vi "Measurement UI.vi"() -> ()   [LabVIEW 2021, in "Load Transient Response_PMIC.lvlib"]
uses:
  Load Transient Response_PMIC.lvlib
panel:
  in  "MeasGraphs":enum32{"LOAD TRANSIENT", "Hidden Controls"}(tab)
  out "MeasTable":string[][](table)
  out "LoadCurrentV/STimeGraph":waveform(dbl)(graph) caption="Load Transient"
  out "OutputVoltageV/STimeGraph":waveform(dbl)(graph) caption="Load Transient"
  in  "Load Current v/s Time":string="LOAD CURRENT vs TIME"
  in  "Output Voltage v/s Time":string="LOAD VOLTAGE vs TIME"
  out "Overshoot load voltage":dbl
  out "Undershoot load voltage":dbl
  in  "Source resource name":string
  in  "Load resource name":string
  out "dt":dbl
  out "Load voltages":dbl[](array[numeric])
  out "Load currents":dbl[](array[numeric])
  in  "Source transient response":i32(ring)=1042 items=["Slow"=1041, "Normal"=1038, "Fast"=1039, "Custom"=1042]
  in  "Load transient response":i32(ring)=3 items=["Slow"=1041, "Normal"=1038, "Fast"=1039, "Custom"=1042]
  in  "Load sense":i32(ring)=1009 caption="SENSE" items=["Local"=1008, "Remote"=1009]
  in  "Source sense":i32(ring)=1009 caption="SENSE" items=["Local"=1008, "Remote"=1009]
  in  "Load current delay t2":dbl=0.001 caption="DELAY T2" format="%#_6ps"
  in  "Load current delay t1":dbl=0.001 caption="DELAY T1" format="%#_6ps"
  in  "Load current pulse duration":dbl=0.001 caption="PULSE DURATION" format="%#_6ps"
  in  "Load current level range":dbl=40.0 caption="CURRENT LEVEL RANGE" format="%#_6pA"
  in  "Load current rising slew rate":dbl=24.0 caption="CURRENT RISING SLEW RATE" format="%#_6pA/us"
  in  "Load current falling slew rate":dbl=24.0 caption="CURRENT FALLING SLEW RATE" format="%#_6pA/us"
  in  "Load configuration":string="Load configuration"
  in  "Source configuration":string="Source configuration"
  in  "Source voltage level":dbl=12.0 caption="VOLTAGE LEVEL" format="%#_6pV"
  in  "Source current limit":dbl=25.0 caption="CURRENT LIMIT" format="%#_6pA"
  in  "PPSResourceName":refnum<k15> caption="RESOURCE NAME"
  in  "Source voltage pole-zero ratio":dbl=2.0 caption="POLE-ZERO RATIO"
  in  "Source voltage gain bandwidth":dbl=2000.0 caption="GAIN BANDWIDTH" format="%#_6pHz"
  in  "Source voltage compensation frequency":dbl=3530.0 caption="COMP. FREQUENCY" format="%#_6pHz"
  in  "Source fast":bool
  in  "Source normal":bool
  in  "Source slow":bool
  in  "Source SourceAdapt":string="Voltage SourceAdapt Parameters"
  in  "Load voltage limit range":dbl=6.0 caption="VOLTAGE LIMIT RANGE" format="%#_6pV"
  in  "Load current set point 1":dbl=4.0 caption="CURRENT SET POINT 1" format="%#_6pA"
  in  "Load current pole-zero ratio":dbl=0.3 caption="POLE-ZERO RATIO"
  in  "Load current gain bandwidth":dbl=14000.0 caption="GAIN BANDWIDTH" format="%#_6pHz"
  in  "Load current compensation frequency":dbl=180000.0 caption="COMP. FREQUENCY" format="%#_6pHz"
  in  "Load sample rate":dbl=1800000.0 caption="SAMPLE RATE" format="%#_6pS/s"
  in  "Load current set point 2":dbl=14.0 caption="CURRENT SET POINT 2" format="%#_6pA"
  in  "ELOADResourceName":refnum<k15> caption="RESOURCE NAME"
  in  "Load fast":bool
  in  "Load normal":bool
  in  "Load slow":bool
  in  "Load SourceAdapt":string="Current SourceAdapt Parameters"
  out "Status":string
  in  "DUT setup time":dbl=1.0 caption="DUT SETUP TIME" format="%#_6ps"
  in  "Measurement settings":string="Measurement settings"
  in  "Nominal output voltage":dbl=3.3 caption="NOMINAL OUTPUT VOLTAGE" format="%#_6pV"
  in  "Mode of operation":T1(ring)=enum."Perform measurement" caption="MODE OF OPERATION"
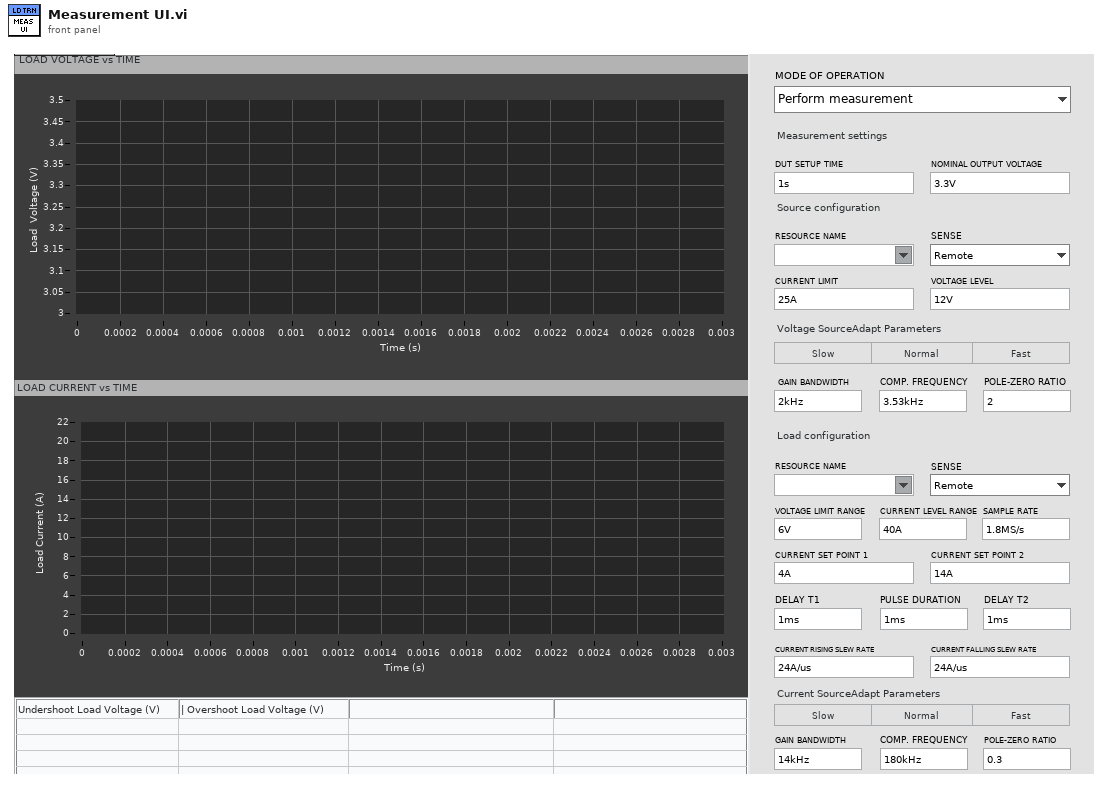
[diagram p1: front panel]
types:
  T1 = enum32{"Power on the DUT", "Perform measurement", "Power off the DUT"}
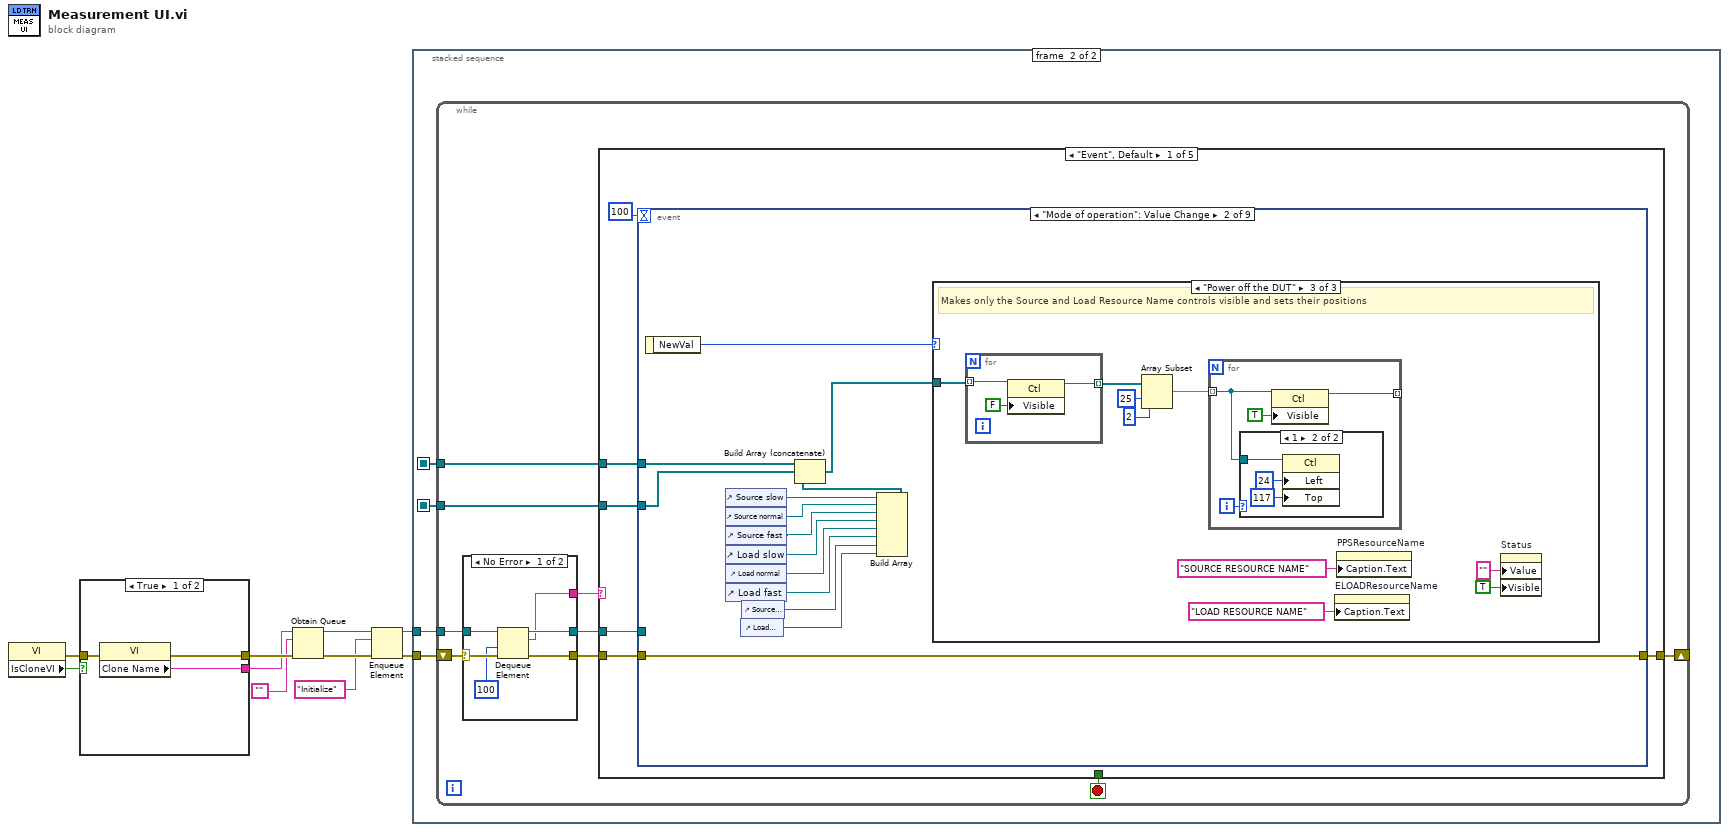
[diagram p0: block diagram]
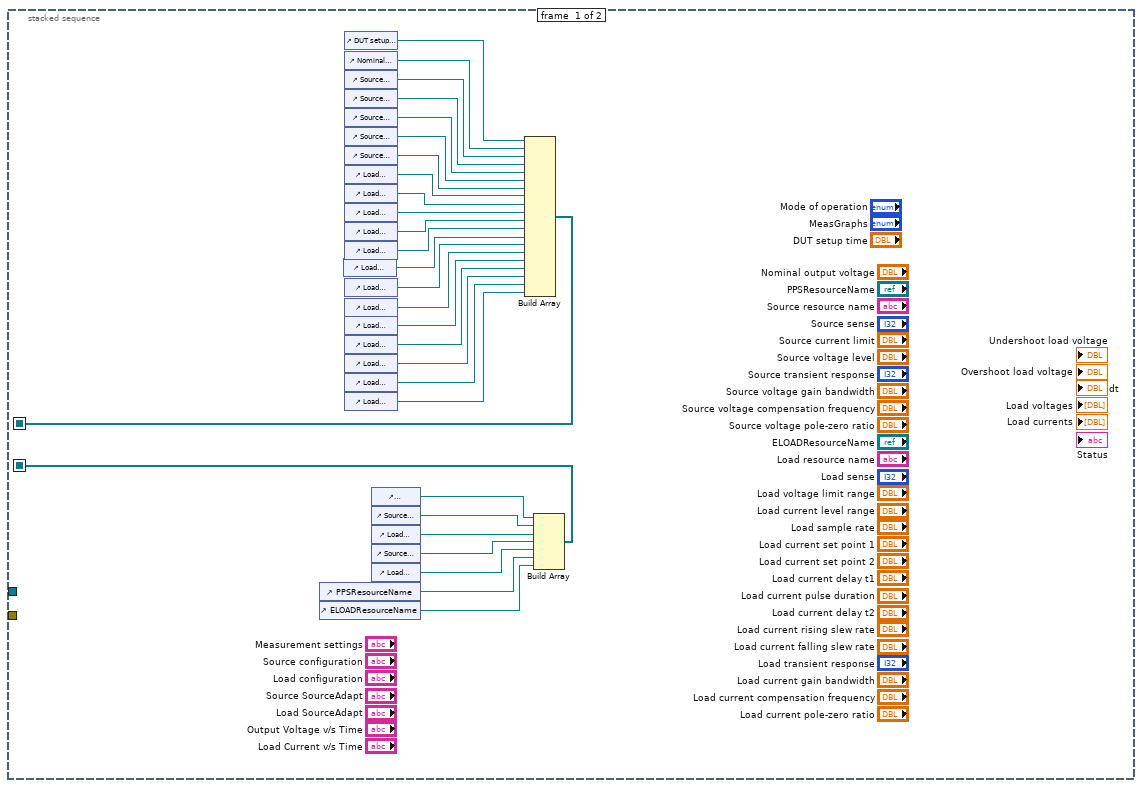
[diagram p2: hidden frame]
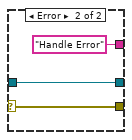
[diagram p3: hidden frame]
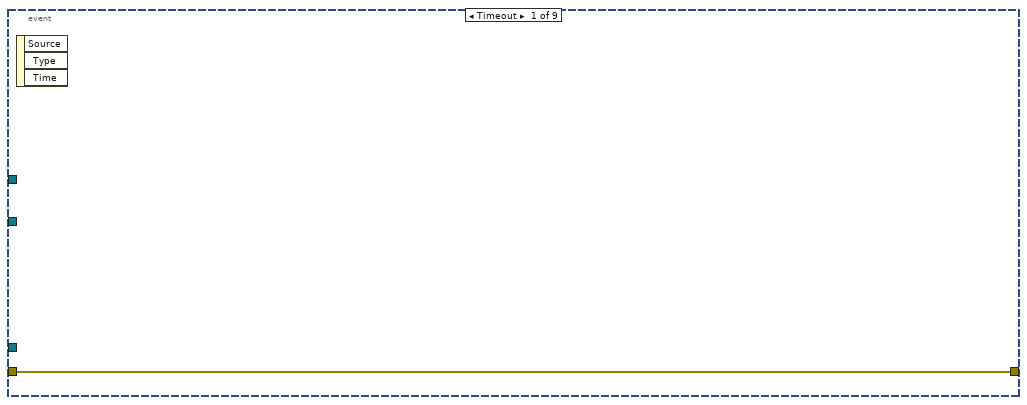
[diagram p4: hidden frame]
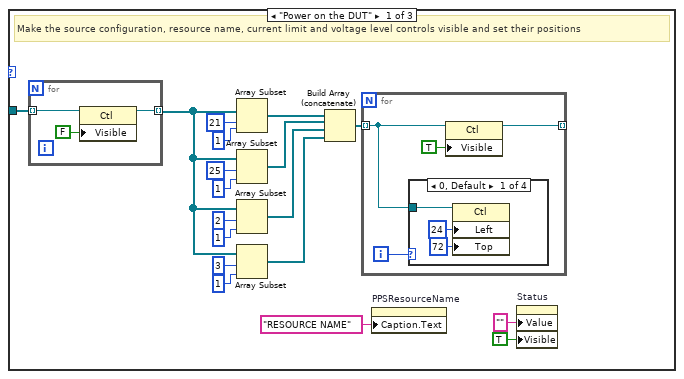
[diagram p5: hidden frame]
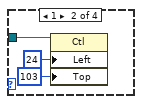
[diagram p6: hidden frame]
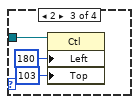
[diagram p7: hidden frame]
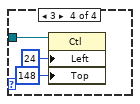
[diagram p8: hidden frame]
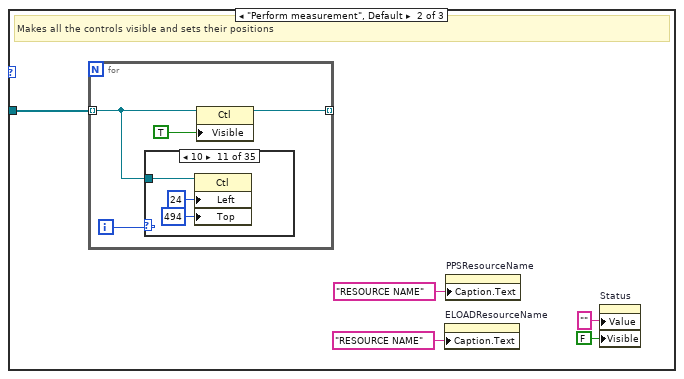
[diagram p9: hidden frame]
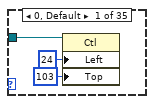
[diagram p10: hidden frame]
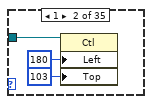
[diagram p11: hidden frame]
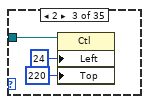
[diagram p12: hidden frame]
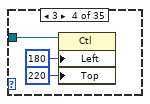
[diagram p13: hidden frame]
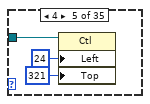
[diagram p14: hidden frame]
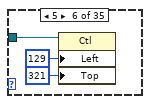
[diagram p15: hidden frame]
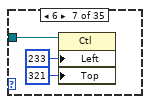
[diagram p16: hidden frame]
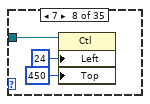
[diagram p17: hidden frame]
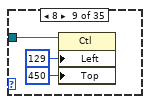
[diagram p18: hidden frame]
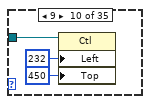
[diagram p19: hidden frame]
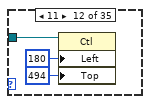
[diagram p20: hidden frame]
diagram:
  n1 = property class="VI"() -> (error out=w1:errorcluster, "IsCloneVI"=w2:bool)  [unwired: 2 in, 1 out]
  n2 = case shown="True" w2 {
    tunnel: [w13 w16] -> w10
    tunnel: [w12 w15] -> w9
    tunnel: w1 -> [w11 w14]
    frame True {
      n3 = property class="VI"(error in=w11) -> (error out=w13:errorcluster, "Clone Name"=w12:string)  [unwired: 1 in, 1 out]
    }
    frame False {
      n4 = property class="VI"(error in=w14) -> (error out=w16:errorcluster, "Name"=w15:string)  [unwired: 1 in, 1 out]
    }
  }
  n5 = Obtain Queue(name (unnamed)=w9, element data type="", error in (no error)=w10) -> (queue out=w6:refnum<queue>, error out=w8:errorcluster)  [unwired: 2 in, 1 out]
  n6 = Enqueue Element(queue=w6, element="Initialize", error in (no error)=w8) -> (queue out=w5:refnum<queue>, error out=w7:errorcluster)  [unwired: 1 in, 1 out]
  n7 = stacked-sequence {
    seq-local: [w29 _] -> [_ w47]
    seq-local: [w30 _] -> [_ w46]
    tunnel: w7 -> [_ w49]
    tunnel: w5 -> [_ w48]
    frame #0 {
      n8 = control-ref of="PPSResourceName"() -> (w33:refnum<vi>)
      n9 = control-ref of="ELOADResourceName"() -> (w34:refnum<vi>)
      n10 = control-ref of="Load current delay t1"() -> (w19:refnum<vi>)
      n11 = control-ref of="DUT setup time"() -> (w22:refnum<vi>)
      n12 = control-ref of="Nominal output voltage"() -> (w45:refnum<vi>)
      n13 = control-ref of="Source current limit"() -> (w44:refnum<vi>)
      n14 = control-ref of="Source voltage level"() -> (w43:refnum<vi>)
      n15 = control-ref of="Source voltage gain bandwidth"() -> (w42:refnum<vi>)
      n16 = control-ref of="Source voltage compensation frequency"() -> (w41:refnum<vi>)
      n17 = control-ref of="Source voltage pole-zero ratio"() -> (w40:refnum<vi>)
      n18 = control-ref of="Load voltage limit range"() -> (w39:refnum<vi>)
      n19 = control-ref of="Load current level range"() -> (w24:refnum<vi>)
      n20 = control-ref of="Load sample rate"() -> (w38:refnum<vi>)
      n21 = control-ref of="Load current set point 1"() -> (w37:refnum<vi>)
      n22 = control-ref of="Load current set point 2"() -> (w36:refnum<vi>)
      n23 = control-ref of="Load current pulse duration"() -> (w18:refnum<vi>)
      n24 = control-ref of="Load current delay t2"() -> (w17:refnum<vi>)
      n25 = control-ref of="Load current rising slew rate"() -> (w20:refnum<vi>)
      n26 = control-ref of="Load current falling slew rate"() -> (w21:refnum<vi>)
      n27 = control-ref of="Load current gain bandwidth"() -> (w23:refnum<vi>)
      n28 = control-ref of="Load current compensation frequency"() -> (w35:refnum<vi>)
      n29 = control-ref of="Load current pole-zero ratio"() -> (w31:refnum<vi>)
      n30 = control-ref of="Measurement settings"() -> (w32:refnum<vi>)
      n31 = control-ref of="Source configuration"() -> (w28:refnum<vi>)
      n32 = control-ref of="Load configuration"() -> (w27:refnum<vi>)
      n33 = control-ref of="Source SourceAdapt"() -> (w26:refnum<vi>)
      n34 = control-ref of="Load SourceAdapt"() -> (w25:refnum<vi>)
      n35 = Build Array(w22, w45, w44, w43, w42, w41, w40, w39, w24, w38, w37, w36, w19, w18, w17, w20, w21, w23, w35, w31) -> (w29:refnum<vi>[])
      n36 = Build Array(w32, w28, w27, w26, w25, w33, w34) -> (w30:refnum<vi>[])
    }
    frame #1 {
      n37 = while {
        shift-right: [w53] -> _
        shift-left: w49 -> [w58]
        tunnel: w48 -> [w56]
        tunnel: w47 -> [w51]
        tunnel: w46 -> [w50]
        stop <- w52 stop-if-true
        n38 = case shown="No Error" w58 {
          selector: w58 -> [w64 w67]
          tunnel: [w63 w67] -> w57
          tunnel: w56 -> [w62 w66]
          tunnel: [w61 w66] -> w55
          tunnel: [w60 "Handle Error"] -> w54
          frame No Error {
            n39 = Dequeue Element(queue=w62, timeout in ms (-1)=100, error in (no error)=w64) -> (queue out=w61:refnum<queue>, element=w60:string, error out=w63:errorcluster)  [unwired: 1 out]
          }
          frame Error {
          }
        }
        n40 = case shown="\"Event\", Default" w54 {
          tunnel: w57 -> [w72 w313 w327 w339 w340]
          tunnel: w55 -> [w70 _ _ w337 _]
          tunnel: [w73 w313 w327 w328 w340] -> w53
          tunnel: [_ FALSE _ TRUE _] -> w52
          tunnel: w51 -> [w69 _ _ w333 _]
          tunnel: w50 -> [w68 _ _ w332 _]
          frame "Event", Default {
            n41 = event shown="[1] \"Mode of operation\": Value Change" {
              selector: _ -> [_ _ _ _ _ _ _ _ _]
              dyn-events: _ -> [_ _ _ _ _ _ _ _ _]
              timeout: 100 -> [_ _ _ _ _ _ _ _ _]
              tunnel: [w74 w84 w262 w264 _ _ _ _ w306] -> w73
              tunnel: w72 -> [w74 w84 w262 w264 _ _ _ _ w307]
              tunnel: w70 -> [_ _ _ _ _ _ _ _ w305]
              tunnel: w69 -> [_ w86 _ _ _ _ _ _ _]
              tunnel: w68 -> [_ w85 _ _ _ _ _ _ _]
              event Timeout {
                n42 = event-data() -> ()  [unwired: 1 in, 3 out]
              }
              event "Mode of operation": Value Change {
                n43 = event-data() -> ("NewVal"=w88:T1)  [unwired: 1 in]
                n44 = control-ref of="Source slow"() -> (w83:refnum<vi>)
                n45 = control-ref of="Source normal"() -> (w82:refnum<vi>)
                n46 = control-ref of="Source fast"() -> (w78:refnum<vi>)
                n47 = control-ref of="Load slow"() -> (w81:refnum<vi>)
                n48 = control-ref of="Load normal"() -> (w80:refnum<vi>)
                n49 = control-ref of="Load fast"() -> (w79:refnum<vi>)
                n50 = control-ref of="Load sense"() -> (w75:refnum<vi>)
                n51 = control-ref of="Source sense"() -> (w76:refnum<vi>)
                n52 = Build Array(w83, w82, w78, w81, w80, w79, w76, w75) -> (w77:refnum<vi>[])
                n53 = Build Array (concatenate)(w86, w85, w77) -> (w87:refnum<vi>[])
                n54 = case shown="\"Power off the DUT\"" w88 {
                  tunnel: w87 -> [w92 w130 w244]
                  frame "Power on the DUT" {
                    # "Make the source configuration, resource name, current limit and voltage level controls visible and set their positions"
                    n55 = for {
                      tunnel: w92 -> [w109] mode=indexing
                      tunnel: [w107] -> w103 mode=indexing
                      n56 = property class="Ctl"(reference=w109, "Visible"=FALSE) -> (reference out=w107:refnum<vi>)  [unwired: 1 in, 1 out]
                    }
                    n57 = Array Subset(array=w103, index=21 ("length"), length=1 ("index")) -> (w101:refnum<vi>[])
                    n58 = Array Subset(array=w103, index=25 ("length"), length=1 ("index")) -> (w102:refnum<vi>[])
                    n59 = Array Subset(array=w103, index=2 ("length"), length=1 ("index")) -> (w104:refnum<vi>[])
                    n60 = Array Subset(array=w103, index=3 ("length"), length=1 ("index")) -> (w106:refnum<vi>[])
                    n61 = Build Array (concatenate)(w101, w102, w104, w106) -> (w105:refnum<vi>[])
                    n62 = for {
                      tunnel: [w112] -> _ mode=indexing
                      tunnel: w105 -> [w110] mode=indexing
                      i -> [w111]
                      n63 = case shown="0, Default" w111 {
                        tunnel: w110 -> [w116 w119 w122 w125]
                        frame 0, Default {
                          n64 = property class="Ctl"(reference=w116, "Left"=24 ("Position:Left"), "Top"=72 ("Position:Top")) -> ()  [unwired: 1 in, 2 out]
                        }
                        frame 1 {
                          n65 = property class="Ctl"(reference=w119, "Left"=24 ("Position:Left"), "Top"=103 ("Position:Top")) -> ()  [unwired: 1 in, 2 out]
                        }
                        frame 2 {
                          n66 = property class="Ctl"(reference=w122, "Left"=180 ("Position:Left"), "Top"=103 ("Position:Top")) -> ()  [unwired: 1 in, 2 out]
                        }
                        frame 3 {
                          n67 = property class="Ctl"(reference=w125, "Left"=24 ("Position:Left"), "Top"=148 ("Position:Top")) -> ()  [unwired: 1 in, 2 out]
                        }
                      }
                      n68 = property class="Ctl"(reference=w110, "Visible"=TRUE) -> (reference out=w112:refnum<vi>)  [unwired: 1 in, 1 out]
                    }
                    n69 = property on="PPSResourceName" class="IVIName"("Caption.Text"="RESOURCE NAME") -> ()  [unwired: 2 in, 2 out]
                    n70 = property on="Status" class="Str"("Value"="" ("Status"), "Visible"=TRUE) -> ()  [unwired: 2 in, 2 out]
                  }
                  frame "Perform measurement", Default {
                    # "Makes all the controls visible and sets their positions"
                    n71 = for {
                      tunnel: w130 -> [w131] mode=indexing
                      tunnel: [w133] -> _ mode=indexing
                      i -> [w132]
                      n72 = case shown="10" w132 {
                        tunnel: w131 -> [w137 w140 w143 w146 w149 w152 w155 w158 w161 w164 w167 w170 w173 w176 w179 w182 w185 w188 w191 w192 w195 w198 w201 w204 w207 w210 w213 w216 w220 w222 w225 w228 w231 w234 w237]
                        frame 0, Default {
                          n73 = property class="Ctl"(reference=w137, "Left"=24 ("Position:Left"), "Top"=103 ("Position:Top")) -> ()  [unwired: 1 in, 2 out]
                        }
                        frame 1 {
                          n74 = property class="Ctl"(reference=w140, "Left"=180 ("Position:Left"), "Top"=103 ("Position:Top")) -> ()  [unwired: 1 in, 2 out]
                        }
                        frame 2 {
                          n75 = property class="Ctl"(reference=w143, "Left"=24 ("Position:Left"), "Top"=220 ("Position:Top")) -> ()  [unwired: 1 in, 2 out]
                        }
                        frame 3 {
                          n76 = property class="Ctl"(reference=w146, "Left"=180 ("Position:Left"), "Top"=220 ("Position:Top")) -> ()  [unwired: 1 in, 2 out]
                        }
                        frame 4 {
                          n77 = property class="Ctl"(reference=w149, "Left"=24 ("Position:Left"), "Top"=321 ("Position:Top")) -> ()  [unwired: 1 in, 2 out]
                        }
                        frame 5 {
                          n78 = property class="Ctl"(reference=w152, "Left"=129 ("Position:Left"), "Top"=321 ("Position:Top")) -> ()  [unwired: 1 in, 2 out]
                        }
                        frame 6 {
                          n79 = property class="Ctl"(reference=w155, "Left"=233 ("Position:Left"), "Top"=321 ("Position:Top")) -> ()  [unwired: 1 in, 2 out]
                        }
                        frame 7 {
                          n80 = property class="Ctl"(reference=w158, "Left"=24 ("Position:Left"), "Top"=450 ("Position:Top")) -> ()  [unwired: 1 in, 2 out]
                        }
                        frame 8 {
                          n81 = property class="Ctl"(reference=w161, "Left"=129 ("Position:Left"), "Top"=450 ("Position:Top")) -> ()  [unwired: 1 in, 2 out]
                        }
                        frame 9 {
                          n82 = property class="Ctl"(reference=w164, "Left"=232 ("Position:Left"), "Top"=450 ("Position:Top")) -> ()  [unwired: 1 in, 2 out]
                        }
                        frame 10 {
                          n83 = property class="Ctl"(reference=w167, "Left"=24 ("Position:Left"), "Top"=494 ("Position:Top")) -> ()  [unwired: 1 in, 2 out]
                        }
                        frame 11 {
                          n84 = property class="Ctl"(reference=w170, "Left"=180 ("Position:Left"), "Top"=494 ("Position:Top")) -> ()  [unwired: 1 in, 2 out]
                        }
                        frame 12 {
                          n85 = property class="Ctl"(reference=w173, "Left"=24 ("Position:Left"), "Top"=539 ("Position:Top")) -> ()  [unwired: 1 in, 2 out]
                        }
                        frame 13 {
                          n86 = property class="Ctl"(reference=w176, "Left"=129 ("Position:Left"), "Top"=539 ("Position:Top")) -> ()  [unwired: 1 in, 2 out]
                        }
                        frame 14 {
                          n87 = property class="Ctl"(reference=w179, "Left"=233 ("Position:Left"), "Top"=539 ("Position:Top")) -> ()  [unwired: 1 in, 2 out]
                        }
                        frame 15 {
                          n88 = property class="Ctl"(reference=w182, "Left"=24 ("Position:Left"), "Top"=588 ("Position:Top")) -> ()  [unwired: 1 in, 2 out]
                        }
                        frame 16 {
                          n89 = property class="Ctl"(reference=w185, "Left"=180 ("Position:Left"), "Top"=588 ("Position:Top")) -> ()  [unwired: 1 in, 2 out]
                        }
                        frame 17 {
                          n90 = property class="Ctl"(reference=w188, "Left"=24 ("Position:Left"), "Top"=679 ("Position:Top")) -> ()  [unwired: 1 in, 2 out]
                        }
                        frame 18 {
                          n91 = property class="Ctl"(reference=w191, "Left"=129 ("Position:Left"), "Top"=679 ("Position:Top")) -> ()  [unwired: 1 in, 2 out]
                        }
                        frame 19 {
                          n92 = property class="Ctl"(reference=w192, "Left"=233 ("Position:Left"), "Top"=679 ("Position:Top")) -> ()  [unwired: 1 in, 2 out]
                        }
                        frame 20 {
                          n93 = property class="Ctl"(reference=w195, "Left"=24 ("Position:Left"), "Top"=72 ("Position:Top")) -> ()  [unwired: 1 in, 2 out]
                        }
                        frame 21 {
                          n94 = property class="Ctl"(reference=w198, "Left"=24 ("Position:Left"), "Top"=144 ("Position:Top")) -> ()  [unwired: 1 in, 2 out]
                        }
                        frame 22 {
                          n95 = property class="Ctl"(reference=w201, "Left"=24 ("Position:Left"), "Top"=372 ("Position:Top")) -> ()  [unwired: 1 in, 2 out]
                        }
                        frame 23 {
                          n96 = property class="Ctl"(reference=w204, "Left"=24 ("Position:Left"), "Top"=264 ("Position:Top")) -> ()  [unwired: 1 in, 2 out]
                        }
                        frame 24 {
                          n97 = property class="Ctl"(reference=w207, "Left"=24 ("Position:Left"), "Top"=630 ("Position:Top")) -> ()  [unwired: 1 in, 2 out]
                        }
                        frame 25 {
                          n98 = property class="Ctl"(reference=w210, "Left"=24 ("Position:Left"), "Top"=175 ("Position:Top")) -> ()  [unwired: 1 in, 2 out]
                        }
                        frame 26 {
                          n99 = property class="Ctl"(reference=w213, "Left"=24 ("Position:Left"), "Top"=405 ("Position:Top")) -> ()  [unwired: 1 in, 2 out]
                        }
                        frame 27 {
                          n100 = property class="Ctl"(reference=w216, "Left"=24 ("Position:Left"), "Top"=288 ("Position:Top")) -> ()  [unwired: 1 in, 2 out]
                        }
                        frame 28 {
                          n101 = property class="Ctl"(reference=w220, "Left"=121 ("Position:Left"), "Top"=288 ("Position:Top")) -> ()  [unwired: 1 in, 2 out]
                        }
                        frame 29 {
                          n102 = property class="Ctl"(reference=w222, "Left"=222 ("Position:Left"), "Top"=288 ("Position:Top")) -> ()  [unwired: 1 in, 2 out]
                        }
                        frame 30 {
                          n103 = property class="Ctl"(reference=w225, "Left"=24 ("Position:Left"), "Top"=650 ("Position:Top")) -> ()  [unwired: 1 in, 2 out]
                        }
                        frame 31 {
                          n104 = property class="Ctl"(reference=w228, "Left"=121 ("Position:Left"), "Top"=650 ("Position:Top")) -> ()  [unwired: 1 in, 2 out]
                        }
                        frame 32 {
                          n105 = property class="Ctl"(reference=w231, "Left"=222 ("Position:Left"), "Top"=650 ("Position:Top")) -> ()  [unwired: 1 in, 2 out]
                        }
                        frame 33 {
                          n106 = property class="Ctl"(reference=w234, "Left"=180 ("Position:Left"), "Top"=175 ("Position:Top")) -> ()  [unwired: 1 in, 2 out]
                        }
                        frame 34 {
                          n107 = property class="Ctl"(reference=w237, "Left"=180 ("Position:Left"), "Top"=405 ("Position:Top")) -> ()  [unwired: 1 in, 2 out]
                        }
                      }
                      n108 = property class="Ctl"(reference=w131, "Visible"=TRUE) -> (reference out=w133:refnum<vi>)  [unwired: 1 in, 1 out]
                    }
                    n109 = property on="ELOADResourceName" class="IVIName"("Caption.Text"="RESOURCE NAME") -> ()  [unwired: 2 in, 2 out]
                    n110 = property on="PPSResourceName" class="IVIName"("Caption.Text"="RESOURCE NAME") -> ()  [unwired: 2 in, 2 out]
                    n111 = property on="Status" class="Str"("Value"="" ("Operation"), "Visible"=FALSE) -> ()  [unwired: 2 in, 2 out]
                  }
                  frame "Power off the DUT" {
                    # "Makes only the Source and Load Resource Name controls visible and sets their positions"
                    n112 = for {
                      tunnel: w244 -> [w250] mode=indexing
                      tunnel: [w249] -> w248 mode=indexing
                      n113 = property class="Ctl"(reference=w250, "Visible"=FALSE) -> (reference out=w249:refnum<vi>)  [unwired: 1 in, 1 out]
                    }
                    n114 = Array Subset(array=w248, index=25 ("length"), length=2 ("index")) -> (w247:refnum<vi>[])
                    n115 = for {
                      tunnel: w247 -> [w252] mode=indexing
                      tunnel: [w254] -> _ mode=indexing
                      i -> [w253]
                      n116 = case shown="1" w253 {
                        tunnel: w252 -> [w258 w261]
                        frame 0, Default {
                          n117 = property class="Ctl"(reference=w258, "Left"=24 ("Position:Left"), "Top"=72 ("Position:Top")) -> ()  [unwired: 1 in, 2 out]
                        }
                        frame 1 {
                          n118 = property class="Ctl"(reference=w261, "Left"=24 ("Position:Left"), "Top"=117 ("Position:Top")) -> ()  [unwired: 1 in, 2 out]
                        }
                      }
                      n119 = property class="Ctl"(reference=w252, "Visible"=TRUE) -> (reference out=w254:refnum<vi>)  [unwired: 1 in, 1 out]
                    }
                    n120 = property on="ELOADResourceName" class="IVIName"("Caption.Text"="LOAD RESOURCE NAME") -> ()  [unwired: 2 in, 2 out]
                    n121 = property on="PPSResourceName" class="IVIName"("Caption.Text"="SOURCE RESOURCE NAME") -> ()  [unwired: 2 in, 2 out]
                    n122 = property on="Status" class="Str"("Value"="" ("Status"), "Visible"=TRUE) -> ()  [unwired: 2 in, 2 out]
                  }
                }
              }
              event "PPSResourceName": Value Change {
                n123 = event-data() -> ()  [unwired: 1 in, 6 out]
                n124 = property on="PPSResourceName" class="IVIName"() -> ("Value"=w263:refnum<k15>)  [unwired: 2 in, 2 out]
                n125 = property on="Source resource name" class="Str"("Value"=w263) -> ()  [unwired: 2 in, 2 out]
              }
              event "ELOADResourceName": Value Change {
                n126 = event-data() -> ()  [unwired: 1 in, 6 out]
                n127 = property on="ELOADResourceName" class="IVIName"() -> ("Value"=w265:refnum<k15>)  [unwired: 2 in, 2 out]
                n128 = property on="Load resource name" class="Str"("Value"=w265) -> ()  [unwired: 2 in, 2 out]
              }
              event "Source slow", "Source normal", "Source fast": Value Change {
                n129 = event-data() -> ("CtlRef"=w271:refnum<vi>)  [unwired: 1 in]
                n130 = property class="Bool"(reference=w271) -> ("Label.Text"=w270:string)  [unwired: 1 in, 2 out]
                n131 = case shown="\"Source fast\"" w270 {
                  tunnel: [w275 w279 w283] -> w269
                  tunnel: [500.0 ("Source voltage gain bandwidth") 2000.0 ("Source voltage gain bandwidth") 4000.0 ("Source voltage gain bandwidth")] -> w268
                  tunnel: [1120.0 ("Source voltage compensation frequency") 3530.0 ("Source voltage compensation frequency") 11300.0 ("Source voltage compensation frequency")] -> w267
                  tunnel: [5.0 ("Source voltage pole-zero ratio") 2.0 ("Source voltage pole-zero ratio") 1.5 ("Source voltage pole-zero ratio")] -> w266
                  frame "Source slow" {
                    w275 = 1041 items=["Slow"=1041, "Normal"=1038, "Fast"=1039, "Custom"=1042] ("Source transient response")
                  }
                  frame "Source normal", Default {
                    w279 = 1038 items=["Slow"=1041, "Normal"=1038, "Fast"=1039, "Custom"=1042] ("Source transient response")
                  }
                  frame "Source fast" {
                    w283 = 1039 items=["Slow"=1041, "Normal"=1038, "Fast"=1039, "Custom"=1042] ("Source transient response")
                  }
                }
                n132 = property on="Source transient response" class="Ring (strict)"("Value"=w269) -> ()  [unwired: 2 in, 2 out]
                n133 = property on="Source voltage gain bandwidth" class="DigNum (strict)"("Value"=w268) -> ()  [unwired: 2 in, 2 out]
                n134 = property on="Source voltage compensation frequency" class="DigNum (strict)"("Value"=w267) -> ()  [unwired: 2 in, 2 out]
                n135 = property on="Source voltage pole-zero ratio" class="DigNum (strict)"("Value"=w266) -> ()  [unwired: 2 in, 2 out]
              }
              event "Source voltage gain bandwidth", "Source voltage compensation frequency", "Source voltage pole-zero ratio": Value Change {
                w284 = 1042 items=["Slow"=1041, "Normal"=1038, "Fast"=1039, "Custom"=1042] ("Source transient response")
                n136 = event-data() -> ()  [unwired: 1 in, 1 out]
                n137 = property on="Source transient response" class="Ring (strict)"("Value"=w284) -> ()  [unwired: 2 in, 2 out]
              }
              event "Load slow", "Load normal", "Load fast": Value Change {
                n138 = event-data() -> ("CtlRef"=w289:refnum<vi>)  [unwired: 1 in]
                n139 = property class="Bool"(reference=w289) -> ("Label.Text"=w290:string)  [unwired: 1 in, 2 out]
                n140 = case shown="\"Load normal\", Default" w290 {
                  tunnel: [w294 w298 w302] -> w288
                  tunnel: [300.0 ("Load current gain bandwidth") 4000.0 ("Load current gain bandwidth") 14000.0 ("Load current gain bandwidth")] -> w287
                  tunnel: [1500.0 ("Load current compensation frequency") 25000.0 ("Load current compensation frequency") 180000.0 ("Load current compensation frequency")] -> w286
                  tunnel: [0.3 ("Load current pole-zero ratio") 6.0 ("Load current pole-zero ratio") 0.3 ("Load current pole-zero ratio")] -> w285
                  frame "Load slow" {
                    w294 = 1041 items=["Slow"=1041, "Normal"=1038, "Fast"=1039, "Custom"=1042] ("Source transient response")
                  }
                  frame "Load normal", Default {
                    w298 = 1038 items=["Slow"=1041, "Normal"=1038, "Fast"=1039, "Custom"=1042] ("Source transient response")
                  }
                  frame "Load fast" {
                    w302 = 1039 items=["Slow"=1041, "Normal"=1038, "Fast"=1039, "Custom"=1042] ("Source transient response")
                  }
                }
                n141 = property on="Load transient response" class="Ring (strict)"("Value"=w288) -> ()  [unwired: 2 in, 2 out]
                n142 = property on="Load current gain bandwidth" class="DigNum (strict)"("Value"=w287) -> ()  [unwired: 2 in, 2 out]
                n143 = property on="Load current compensation frequency" class="DigNum (strict)"("Value"=w286) -> ()  [unwired: 2 in, 2 out]
                n144 = property on="Load current pole-zero ratio" class="DigNum (strict)"("Value"=w285) -> ()  [unwired: 2 in, 2 out]
              }
              event "Load current gain bandwidth", "Load current compensation frequency", "Load current pole-zero ratio": Value Change {
                w303 = 1042 items=["Slow"=1041, "Normal"=1038, "Fast"=1039, "Custom"=1042] ("Load transient response")
                n145 = event-data() -> ()  [unwired: 1 in, 1 out]
                n146 = property on="Load transient response" class="Ring (strict)"("Value"=w303) -> ()  [unwired: 2 in, 2 out]
              }
              event Panel Close? {
                n147 = event-data() -> ()  [unwired: 1 in, 4 out]
                n148 = Enqueue Element(queue=w305, element="Exit", error in (no error)=w307) -> (error out=w306:errorcluster)  [unwired: 1 in, 2 out]
                n149 = event-data("Discard?"=TRUE) -> ()  [unwired: 1 in, 1 out]
              }
            }
          }
          frame "Initialize" {
            w310 = 2 ("Palette:Active Tool")
            w311 = "<Select Device>"
            n150 = property on="OutputVoltageV/STimeGraph" class="WFGraph (strict)"("ActPaletteTool"=w310) -> ()  [unwired: 2 in, 2 out]
            n151 = property on="PPSResourceName" class="IVIName"("Value"=w311) -> ()  [unwired: 2 in, 2 out]
            n152 = property on="ELOADResourceName" class="IVIName"("Value"=w311) -> ()  [unwired: 2 in, 2 out]
            n153 = property on="LoadCurrentV/STimeGraph" class="WFGraph (strict)"("ActPaletteTool"=w310) -> ()  [unwired: 2 in, 2 out]
            n154 = property on="Status" class="Str"("Visible"=FALSE) -> ()  [unwired: 2 in, 2 out]
          }
          frame "Post UI Update" {
            w318 = "%.3f" ("initial string")
            # "This case will be triggered, after framework updates the User interface with result values."
            n155 = local read "Load voltages"() -> (w324:dbl[])
            n156 = local read "Load currents"() -> (w323:dbl[])
            n157 = local read "dt"() -> (w322:dbl)
            n158 = local read "Undershoot load voltage"() -> (w317:dbl)
            n159 = local read "Overshoot load voltage"() -> (w316:dbl)
            n160 = Bundle By Name("Y"=w324, "dt"=w322) -> (→"OutputVoltageV/STimeGraph":waveform(dbl))  [unwired: 1 in]
            n161 = Bundle By Name("dt"=w322, "Y"=w323) -> (→"LoadCurrentV/STimeGraph":waveform(dbl))  [unwired: 1 in]
            n162 = Format Into String(format string=w318, w317) -> (resulting string=w315:string)  [unwired: 2 in, 1 out]
            n163 = Format Into String(format string=w318, initial string="|   ", w316) -> (resulting string=w314:string)  [unwired: 1 in, 1 out]
            n164 = Build Array(w315, w314) -> (w320:string[])
            n165 = Build Array(w320) -> (→"MeasTable":string[][])
          }
          frame "Exit" {
            # "This case is triggered to close the User Interface from framework"
            n166 = Build Array (concatenate)(w333, w332) -> (w331:refnum<vi>[])
            n167 = Close Reference(reference=w331) -> (error out=w329:errorcluster)  [unwired: 1 in]
            n168 = Flush Queue(queue=w337, error in (no error)=w339) -> (queue out=w336:refnum<queue>, error out=w335:errorcluster)  [unwired: 1 out]
            n169 = Release Queue(queue=w336, force destroy? (F)=TRUE, error in (no error)=w335) -> (error out=w330:errorcluster)  [unwired: 2 out]
            n170 = Merge Errors(w329, w330) -> (w328:errorcluster)
          }
          frame "Handle Error" {
          }
        }
      }
    }
  }
